vi "NR Change Band Status.vi"(7 "Operation Band":u32, 8 "error in (no error)":errorcluster caption="에러 입력(에러 없음)", 9 "BW (MHz)":u32, 10 "Center Channel Number":u32, 11 "Instrument Manager 입력":refnum<class "Instrument Manager.lvclass">) -> (0 "error out":errorcluster caption="에러 출력", 3 "Instrument Manager 출력":refnum<class "Instrument Manager.lvclass">)   [LabVIEW 2023, in "Instrument Manager.lvclass"]
uses:
  Instrument Manager.lvclass
  Module/ANRITSU Call Box/Type Definition/NR Selected CC Type Arguments.ctl
  Instrument Manager.lvclass/Instrument Manager.ctl
  Module/ANRITSU Call Box/Interface Class/Anritsu Call Box.lvclass
  Module/ANRITSU Call Box/ANRITSU Call Box.lvlib
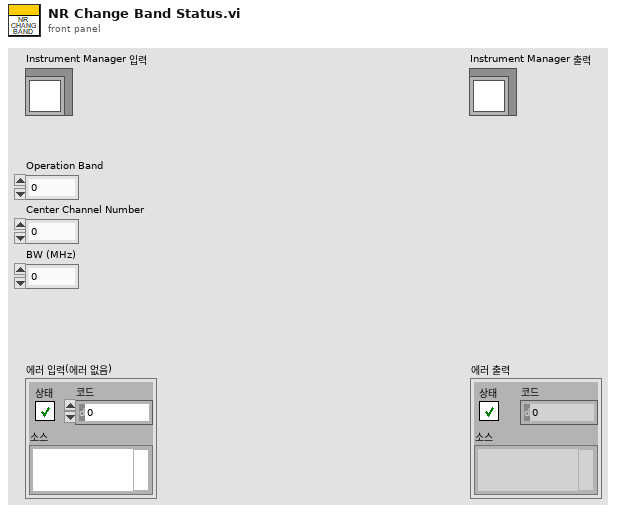
[diagram p1: front panel]
types:
  T1 = typedef "ANRITSU Call Box.lvlib/NR Selected CC Type Arguments.ctl" = cluster{"Selected CC":enum16{"PCC", "SCC", "FR2_PCC", "FR2_SCC"}, "SCC or FR2_SCC Index":u32}
  T2 = cluster{"Anritsu Call Box":refnum<class "Anritsu Call Box.lvclass">, "Spectrum Analyzer":refnum<class "Interface_Spectrum.lvclass">, "RF Switch Box":refnum<class "RF Filter Box.lvclass">, "Turn Table":refnum<class "Interface - Turn Table.lvclass">, "Mast":refnum<class "Interface - Mast.lvclass">, "3D Controller":refnum<class "Interface_3D Controller.lvclass">}
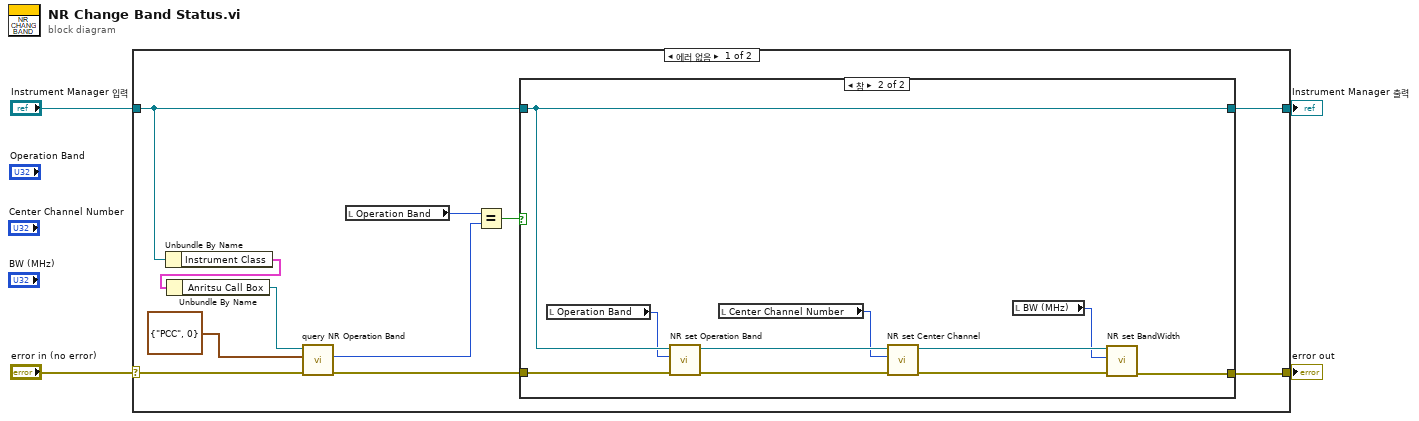
[diagram p0: block diagram]
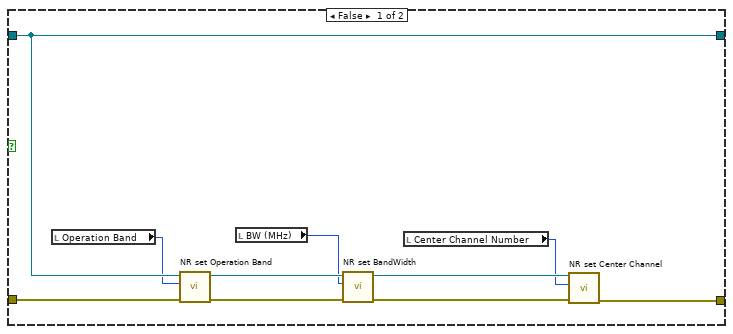
[diagram p2: hidden frame]
diagram:
  n1 = case shown="에러 없음" "error in (no error)" {
    selector: "error in (no error)" -> [w14 w37]
    tunnel: [w10 w37] -> w3
    tunnel: [w8 w36] -> w1
    tunnel: "Instrument Manager 입력" -> [w9 w36]
    frame No Error {
      n2 = Unbundle By Name(w9) -> ("Instrument Class"=w13:T2)
      n3 = Unbundle By Name(w13) -> ("Anritsu Call Box"=w12:refnum<class "Anritsu Call Box.lvclass">)
      n4 = call-dynamic "query NR Operation Band.vi"("error in (no error)"=w14, "Selected CC Argements"=T1 {"Selected CC"=enum."PCC", "SCC or FR2_SCC Index"=0}, "Anritsu Call Box in"=w12) -> ("error out"=w11:errorcluster, "Operation Band"=w7:u32)  [unwired: 6 in, 1 out]
      n5 = local read "Operation Band"() -> (w5:u32)
      n6 = Equal?(x=w5, y=w7) -> (x = y?=w6:bool)
      n7 = case shown="참" w6 {
        tunnel: w11 -> [w25 w35]
        tunnel: [w22 w32] -> w10
        tunnel: w9 -> [w21 w31]
        tunnel: [w21 w31] -> w8
        frame False {
          n8 = local read "Operation Band"() -> (w18:u32)
          n9 = call "NR set Operation Band.vi"("error in (no error)"=w25, "Operation Band"=w18, "Instrument Manager 입력"=w21) -> ("error out"=w24:errorcluster, "Instrument Manager 출력"=w20:refnum<class "Instrument Manager.lvclass">)  [unwired: 7 in]
          n10 = local read "BW (MHz)"() -> (w16:u32)
          n11 = call "NR set BandWidth.vi"("error in (no error)"=w24, "BW (MHz)"=w16, "Instrument Manager 입력"=w20) -> ("error out"=w23:errorcluster, "Instrument Manager 출력"=w19:refnum<class "Instrument Manager.lvclass">)  [unwired: 7 in]
          n12 = local read "Center Channel Number"() -> (w17:u32)
          n13 = call "NR set Center Channel.vi"("error in (no error)"=w23, "Center Channel Number"=w17, "Instrument Manager 입력"=w19) -> ("error out"=w22:errorcluster)  [unwired: 7 in, 1 out]
        }
        frame True {
          n14 = local read "Operation Band"() -> (w28:u32)
          n15 = call "NR set Operation Band.vi"("error in (no error)"=w35, "Operation Band"=w28, "Instrument Manager 입력"=w31) -> ("error out"=w34:errorcluster, "Instrument Manager 출력"=w30:refnum<class "Instrument Manager.lvclass">)  [unwired: 7 in]
          n16 = local read "Center Channel Number"() -> (w27:u32)
          n17 = call "NR set Center Channel.vi"("error in (no error)"=w34, "Center Channel Number"=w27, "Instrument Manager 입력"=w30) -> ("error out"=w33:errorcluster, "Instrument Manager 출력"=w29:refnum<class "Instrument Manager.lvclass">)  [unwired: 7 in]
          n18 = local read "BW (MHz)"() -> (w26:u32)
          n19 = call "NR set BandWidth.vi"("error in (no error)"=w33, "BW (MHz)"=w26, "Instrument Manager 입력"=w29) -> ("error out"=w32:errorcluster)  [unwired: 7 in, 1 out]
        }
      }
    }
    frame Error {
    }
  }
  "error out" <- w3
  "Instrument Manager 출력" <- w1
